vi "Parse Mark Inband.vi"(8 "error in (no error)":errorcluster caption="에러 입력(에러 없음)", 10 "JSON string":string, 11 "Instrument Manager 입력":refnum<class "Instrument Manager.lvclass">) -> (0 "error out":errorcluster caption="에러 출력", 1 "Limit":dbl, 2 "Mark InBand Param":T1, 3 "Instrument Manager 출력":refnum<class "Instrument Manager.lvclass">)   [LabVIEW 2023, in "Instrument Manager.lvclass"]
uses:
  Instrument Manager.lvclass
  Instrument Manager.lvclass/Instrument Manager.ctl
  Param Definition/Mark InBand Param.ctl
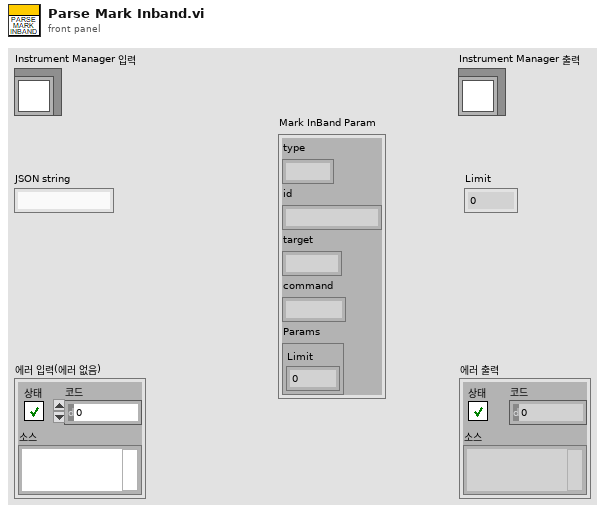
[diagram p1: front panel]
types:
  T1 = typedef "Instrument Manager.lvclass/Mark InBand Param.ctl" = cluster{"type":string, "id":string, "target":string, "command":string, "Params":cluster{"Limit":dbl}}
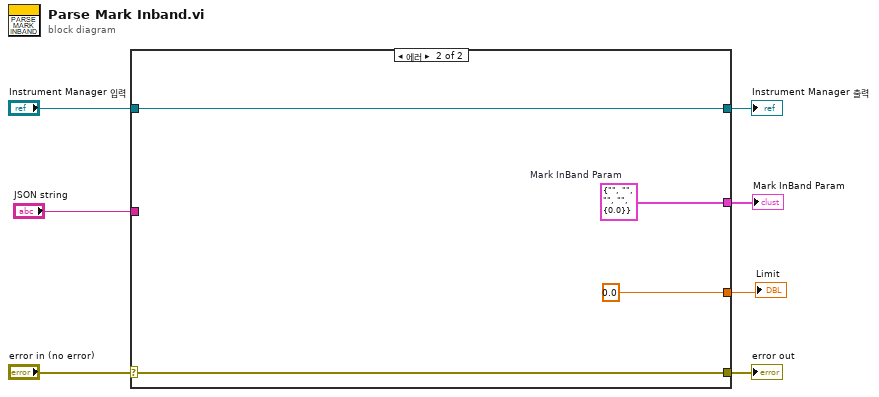
[diagram p0: block diagram]
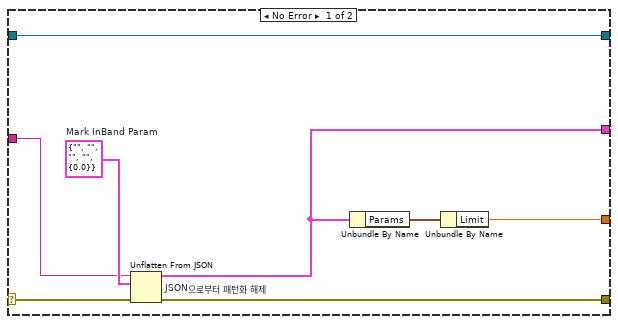
[diagram p2: hidden frame]
diagram:
  n1 = case shown="에러" "error in (no error)" {
    selector: "error in (no error)" -> [w13 w19]
    tunnel: [w12 w19] -> w6
    tunnel: [w15 w18] -> w4
    tunnel: "Instrument Manager 입력" -> [w15 w18]
    tunnel: "JSON string" -> [w11 _]
    tunnel: [w9 0.0 ("Limit")] -> w2
    tunnel: [w8 w17] -> w1
    frame No Error {
      w14 = T1 {"type"="", "id"="", "target"="", "command"="", "Params"={"Limit"=0.0}}  # Mark InBand Param
      n2 = Unflatten From JSON "JSON으로부터 패턴화 해제"(JSON string=w11, type and defaults=w14, error in (no error)=w13) -> (value=w8:T1, error out=w12:errorcluster)  [unwired: 4 in]
      n3 = Unbundle By Name(w8) -> ("Params"=w10:cluster{"Limit":dbl})
      n4 = Unbundle By Name(w10) -> ("Limit"=w9:dbl)
    }
    frame Error {
      w17 = T1 {"type"="", "id"="", "target"="", "command"="", "Params"={"Limit"=0.0}}  # Mark InBand Param
    }
  }
  "error out" <- w6
  "Instrument Manager 출력" <- w4
  "Limit" <- w2
  "Mark InBand Param" <- w1
